vi "File Cleanup.vi"() -> ()   [LabVIEW 2018]
uses:
  7d7c2da0-47d8-4a60-b0ea-b7aa6de509b2.vi
  1757509d-9639-4861-80dd-ee25ca2b0721.vi
  7d7c2da0-47d8-4a60-b0ea-b7aa6de509b2.vi/0a1ee2ab-da6d-4243-8cf3-8125e611a602.vi
  src/api/Log.vi
  src/api/configuration/handlers/file_handler/CleanupFilter.LastMod/CleanupFilter.LastMod.lvclass
  C:/Users/Colin/Documents/software_projects/labview/glog/src/api/configuration/handlers/file_handler/CleanupFilter/CleanupFilter.lvclass
  src/api/configuration/handlers/file_handler/File Handler.lvclass
  C:/Users/Colin/Documents/software_projects/labview/glog/src/api/extension/formatting_handler_interface/Formatting Handler.lvclass
  src/api/configuration/handlers/file_handler/New (Single Trigger).vi
  src/registry/Log.vi
  src/api/GLog.lvlib
panel:
  out "error out":errorcluster
  in  "cleanup?":bool
  out "second file only?":bool
  out "first file created?":bool
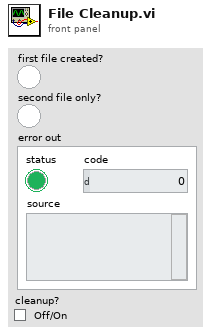
[diagram p1: front panel]
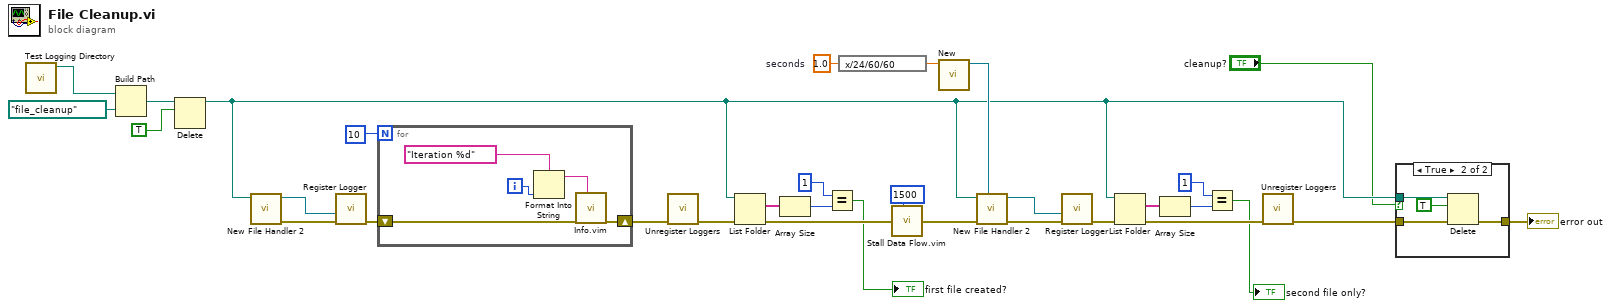
[diagram p0: block diagram]
diagram:
  w31 = 1.0  # seconds
  n1 = call "Test Logging Directory.vi"() -> ("test logging directory"=w20:path)  [unwired: 11 in]
  n2 = Build Path(base path=w20, name or relative path=path "file_cleanup") -> (appended path=w18:path)
  n3 = Delete(path (use dialog)=w18, entire hierarchy (F)=TRUE) -> (deleted path=w3:path)  [unwired: 3 in, 2 out]
  n4 = call-poly "New File Handler 2.vi"("log directory (<app dir>/logs)"=w3) -> ("error out"=w27:errorcluster, "file handler"=w32:refnum<class "File Handler.lvclass">)  [unwired: 8 in, 1 out]
  n5 = call "Register Logger.vi"("error in (no error)"=w27, "log handler (file handler)"=w32) -> ("error out"=w28:errorcluster)  [unwired: 9 in]
  n6 = for {
    N: 10 -> [_]
    shift-right: [w33] -> w26
    shift-left: w28 -> [w33]
    i -> [w34]
    n7 = Format Into String(format string="Iteration %d", w34) -> (resulting string=w36:string)  [unwired: 2 in, 1 out]
    n8 = call "Info.vim"("message"=w36) -> ()  [unwired: 10 in, 1 out]
  }
  n9 = call "Unregister Loggers.vi"("error in (no error)"=w26) -> ("error out"=w15:errorcluster)  [unwired: 9 in, 1 out]
  n10 = List Folder(path=w3, error in=w15) -> (filenames=w13:string[], error out=w14:errorcluster)  [unwired: 2 in, 2 out]
  n11 = Array Size(array=w13) -> (size(s)=w12:i32)
  n12 = Equal?(x=1, y=w12) -> (x = y?=→"first file created?":bool)
  n13 = expression code="x/24/60/60"(w31) -> (w30:dbl)
  n14 = call "Stall Data Flow.vim"("value in"=w14, "milliseconds to wait"=u32 1500) -> ("value out"=w22:errorcluster)  [unwired: 1 out]
  n15 = call "New.vi"("age limit [days](30)"=w30) -> ("Cleanup Filter"=w21:refnum<class "CleanupFilter.LastMod.lvclass">)  [unwired: 10 in]
  n16 = call-poly "New File Handler 2.vi"("cleanup filter (never)"=w21, "error in"=w22, "log directory (<app dir>/logs)"=w3) -> ("error out"=w23:errorcluster, "file handler"=w24:refnum<class "File Handler.lvclass">)  [unwired: 6 in, 1 out]
  n17 = call "Register Logger.vi"("error in (no error)"=w23, "log handler (file handler)"=w24) -> ("error out"=w6:errorcluster)  [unwired: 9 in]
  n18 = List Folder(path=w3, error in=w6) -> (filenames=w9:string[], error out=w5:errorcluster)  [unwired: 2 in, 2 out]
  n19 = Array Size(array=w9) -> (size(s)=w8:i32)
  n20 = Equal?(x=1, y=w8) -> (x = y?=→"second file only?":bool)
  n21 = call "Unregister Loggers.vi"("error in (no error)"=w5) -> ("error out"=w16:errorcluster)  [unwired: 9 in, 1 out]
  n22 = case shown="True" "cleanup?" {
    tunnel: w16 -> [w37 w40]
    tunnel: w3 -> [_ w39]
    tunnel: [w37 w38] -> w1
    frame False {
    }
    frame True {
      n23 = Delete(path (use dialog)=w39, entire hierarchy (F)=TRUE, error in=w40) -> (error out=w38:errorcluster)  [unwired: 2 in, 2 out]
    }
  }
  "error out" <- w1
